vi "Test_TLS.vi"() -> ()   [LabVIEW 2021]
doc: "C5: sends GET /api/version over the C4 TLS connection and reads until the device closes it. Pass = HTTP/1.1 200, “05.00” in the body, and nodelay 1."
uses:
  common/CANsub_Common.lvlib
panel:
  out "error out":errorcluster
  out "pass":bool
  out "response":string
  out "nodelay":i32
  in  "cert path":path=path "/home/lvuser/cansub_root_cert.crt"
  in  "host":string="192.168.0.49"
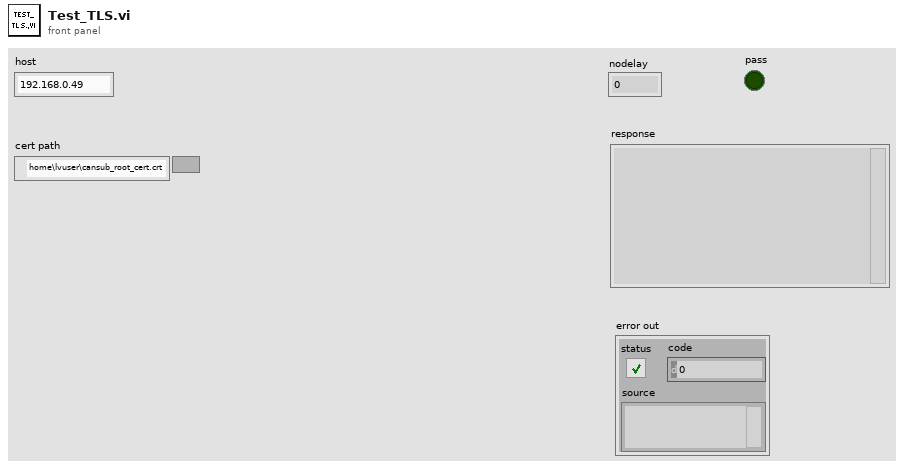
[diagram p1: front panel]
types:
  T1 = enum16{"Standard", "Buffered", "CRLF", "Immediate"}
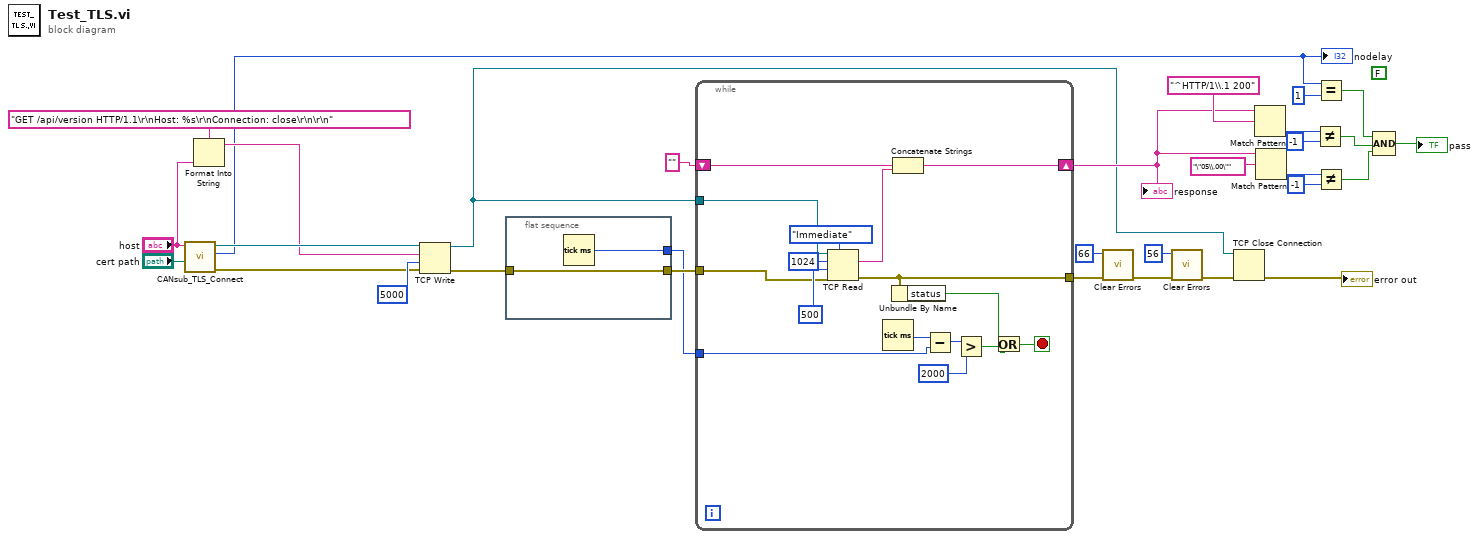
[diagram p0: block diagram]
diagram:
  (unwired) FALSE ("x = y?")
  n1 = call "CANsub_TLS_Connect.vi"("cert path"="cert path", "host"="host") -> ("error out"=w25:errorcluster, "nodelay"=w8:i32, "TLS connection"=w28:refnum<k5>)  [unwired: 7 in]
  "nodelay" <- w8
  n2 = Format Into String(format string="GET /api/version HTTP/1.1\r\nHost: %s\r\nConnection: close\r\n\r\n", "host") -> (resulting string=w27:string)  [unwired: 2 in, 1 out]
  n3 = TCP Write(connection ID=w28, data in=w27, error in (no error)=w25, 9:5000 ("timeout ms (25000)")) -> (connection ID out=w1:refnum<k5>, error out=w24:errorcluster)  [unwired: 1 out]
  n4 = flat-sequence {
    tunnel: w24 -> [w32]
    tunnel: [w33] -> w21
    tunnel: [w32] -> w22
    frame #0 {
      n5 = Tick Count (ms)() -> (millisecond timer value=w33:u32)
    }
  }
  n6 = while {
    shift-right: [w34] -> w3
    shift-left: "" -> [w44]
    tunnel: w1 -> [w46]
    tunnel: w22 -> [w45]
    tunnel: w21 -> [w41]
    tunnel: [w35] -> w20
    stop <- w36 stop-if-true
    n7 = TCP Read(connection ID=w46, bytes to read=1024, error in (no error)=w45, 7:T1."Immediate" ("mode (standard)"), 9:500 ("timeout ms (25000)")) -> (data out=w43:string, error out=w35:errorcluster)  [unwired: 1 out]
    n8 = Tick Count (ms)() -> (millisecond timer value=w42:u32)
    n9 = Unbundle By Name(w35) -> ("status"=w38:bool)
    n10 = Concatenate Strings(w44, w43) -> (w34:string)
    n11 = Subtract(x=w42, y=w41) -> (x-y=w40:u32)
    n12 = Greater?(x=w40, y=u32 2000) -> (0:w37:bool)
    n13 = Or(x=w38, y=w37) -> (x .or. y?=w36:bool)
  }
  "response" <- w3
  n14 = call <vilib>:"Clear Errors.vi"("error in (no error)"=w20, "specific error code to clear (0: all)"=66) -> ("error out"=w19:errorcluster)  [unwired: 4 in, 1 out]
  n15 = call <vilib>:"Clear Errors.vi"("error in (no error)"=w19, "specific error code to clear (0: all)"=56) -> ("error out"=w16:errorcluster)  [unwired: 4 in, 1 out]
  n16 = TCP Close Connection(connection ID=w1, error in (no error)=w16) -> (error out=→"error out":errorcluster)  [unwired: 1 in, 1 out]
  n17 = Match Pattern(string=w3, regular expression="^HTTP/1\\.1 200") -> (offset past match=w13:i32)  [unwired: 1 in, 3 out]
  n18 = Match Pattern(string=w3, regular expression="\"05\\.00\"") -> (offset past match=w9:i32)  [unwired: 1 in, 3 out]
  n19 = Not Equal?(x=w13, y=-1) -> (x != y?=w6:bool)
  n20 = Equal?(x=w8, y=1) -> (x = y?=w5:bool)
  n21 = Not Equal?(x=w9, y=-1) -> (x != y?=w4:bool)
  n22 = Compound Arithmetic op=AND(w5, w6, w4) -> (→"pass":bool)
